vi "Get VI Case Structure Reference.vi"(8 "error in (no error)":errorcluster, 11 "JKI SM in":refnum<class "JKI SM.lvclass">) -> (0 "error out":errorcluster, 2 "Case Structure ref":refnum<vi>, 3 "JKI SM out":refnum<class "JKI SM.lvclass">)   [LabVIEW 2020, in "JKI State Machine API.lvlib" / "JKI SM.lvclass"]
uses:
  JKI SM.lvclass
  JKI SM.lvclass/JKI SM.ctl
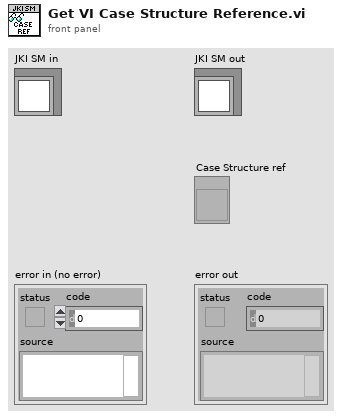
[diagram p1: front panel]
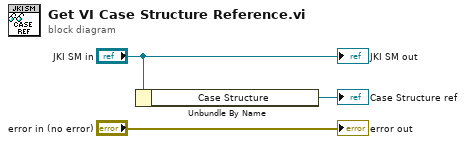
[diagram p0: block diagram]
diagram:
  n1 = Unbundle By Name("JKI SM in") -> ("Case Structure"=→"Case Structure ref":refnum<vi>)
  "error out" <- "error in (no error)"
  "JKI SM out" <- "JKI SM in"
